vi "Fan Params.vi"(8 "error in":errorcluster, 10 "Fan Params Registers":map{string, u16}(c390), 11 "DeepU Results in":refnum<class "DeepU Results.lvclass">) -> (0 "error out":errorcluster, 2 "Fan Const":bool, 3 "DeepU Results out":refnum<class "DeepU Results.lvclass">)   [LabVIEW 2019, in "Results.lvlib" / "DeepU Results.lvclass"]
uses:
  DeepU Results.lvclass
  DeepU Results.lvclass/DeepU Results.ctl
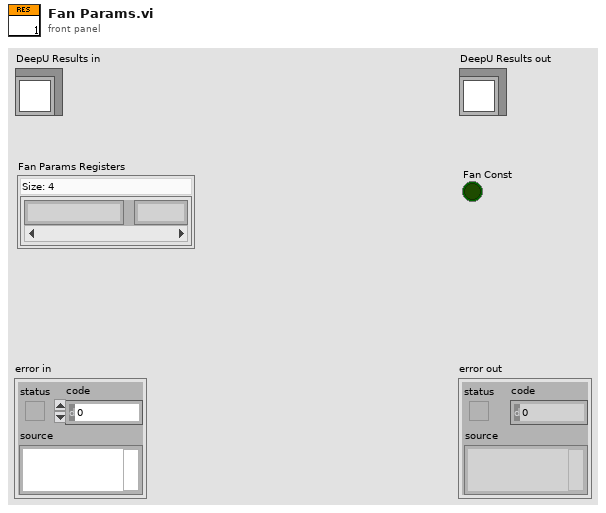
[diagram p1: front panel]
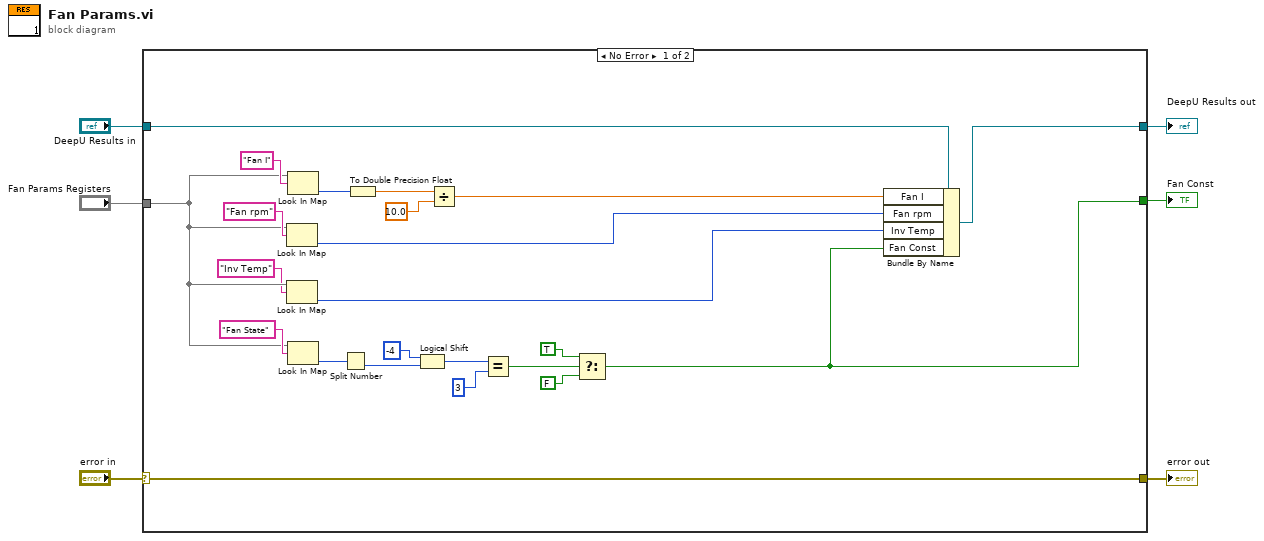
[diagram p0: block diagram]
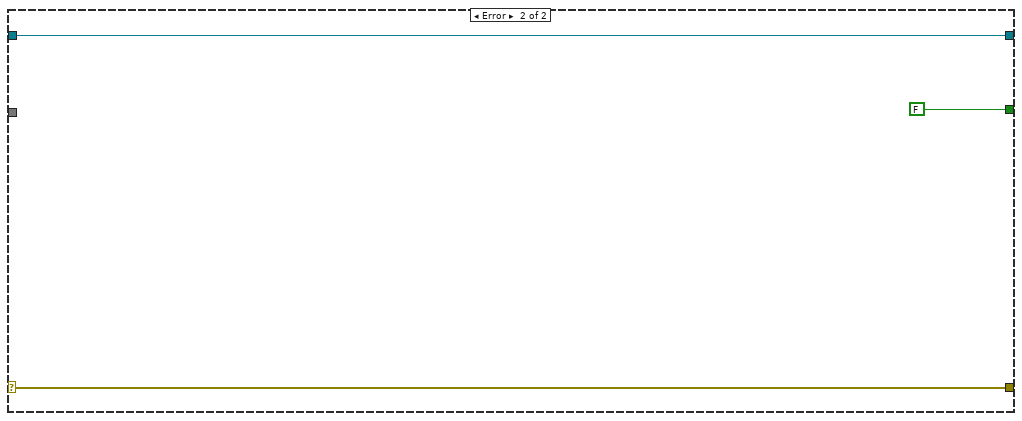
[diagram p2: hidden frame]
diagram:
  n1 = case shown="No Error" "error in" {
    selector: "error in" -> [w28 w32]
    tunnel: [w28 w32] -> w5
    tunnel: [w27 w31] -> w3
    tunnel: "DeepU Results in" -> [w29 w31]
    tunnel: "Fan Params Registers" -> [w23 _]
    tunnel: [w10 FALSE] -> w1
    frame No Error {
      n2 = Look In Map(map=w23, key="Fan rpm") -> (value=w15:u16)  [unwired: 1 in, 1 out]
      n3 = Look In Map(map=w23, key="Inv Temp") -> (value=w16:u16)  [unwired: 1 in, 1 out]
      n4 = Look In Map(map=w23, key="Fan I") -> (value=w14:u16)  [unwired: 1 in, 1 out]
      n5 = Look In Map(map=w23, key="Fan State") -> (value=w8:u16)  [unwired: 1 in, 1 out]
      n6 = Split Number(x=w8) -> (lo(x)=w7:u8)  [unwired: 1 out]
      n7 = To Double Precision Float(number=w14) -> (double precision float=w13:dbl)
      n8 = Logical Shift(y=i16 -4, x=w7) -> (x << y=w9:u8)
      n9 = Divide(x=w13, y=10.0) -> (x/y=w11:dbl)
      n10 = Equal?(x=w9, y=u8 3) -> (x = y?=w19:bool)
      n11 = Select(t=TRUE, s=w19, f=FALSE) -> (s? t:f=w10:bool)
      n12 = Bundle By Name(cluster=w29, "Fan I"=w11, "Fan rpm"=w15, "Inv Temp"=w16, "Fan Const"=w10) -> (w27:refnum<class "DeepU Results.lvclass">)
    }
    frame Error {
    }
  }
  "error out" <- w5
  "DeepU Results out" <- w3
  "Fan Const" <- w1
